vi "Test_Echo_Send_Report.vi"() -> ()   [LabVIEW 2021]
doc: "Test of Echo_Send_Report without device: one stored echo at key 196615, two calls with the same ack. Expect one 36-byte report datagram on 127.0.0.1:report port, TX acks matched 1, unmatched acks 1."
uses:
  echo/Echo_Context.ctl
  echo/Echo_Time_Store.ctl
  echo/Echo_Frame_Kind.ctl
  echo/Echo_Frame.ctl
  echo/Echo_Counters.ctl
panel:
  out "error out":errorcluster
  out "Echo_Counters":T1
  in  "report port":u16=5302
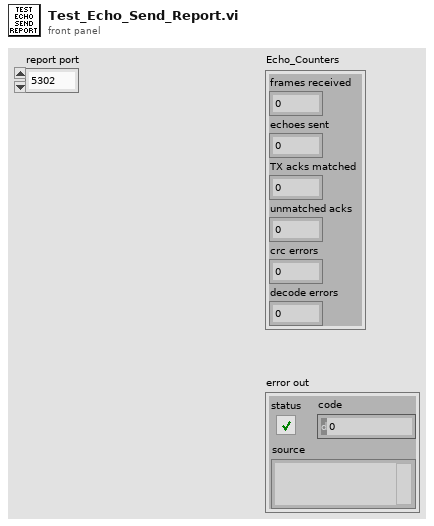
[diagram p1: front panel]
types:
  T1 = typedef "Echo_Counters.ctl" = cluster{"frames received":u32, "echoes sent":u32, "TX acks matched":u32, "unmatched acks":u32, "crc errors":u32, "decode errors":i32}
  T2 = typedef "Echo_Frame_Kind.ctl" = enum16{"Other", "Test", "Ack"}
  T3 = typedef "Echo_Frame.ctl" = cluster{"kind":T2, "id":u32, "t_dev":dbl, "seq":u16, "idx":u8, "key":i32, "index":i32}
  T4 = typedef "Echo_Time_Store.ctl" = cluster{"t_rx2_dev":dbl[], "t_rx2_lv":dbl[], "t_echo_send_lv":dbl[]}
  T5 = typedef "Echo_Context.ctl" = cluster{"TLS connection":refnum<k5>, "udp":refnum<k16>, "lv addr":u32, "report port":u16, "test lo":u32, "test hi":u32, "ack lo":u32, "ack hi":u32, "echo offset":i32}
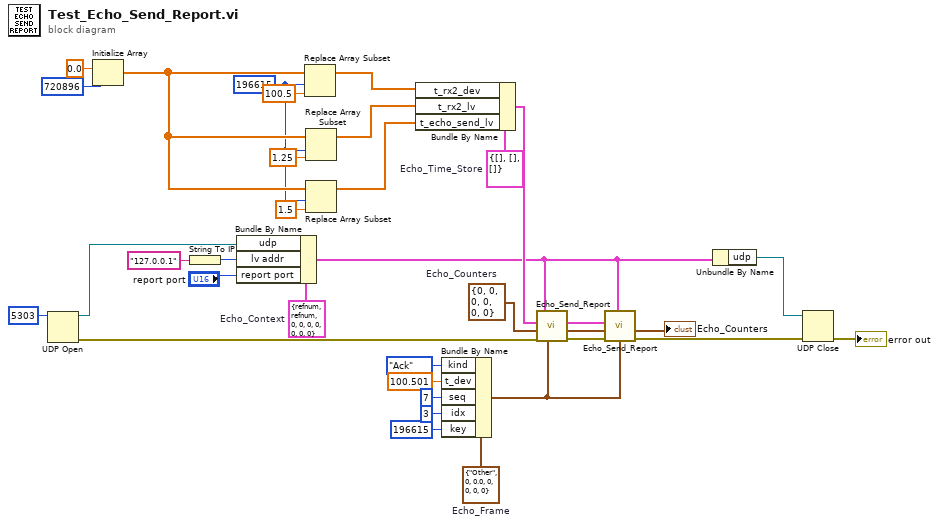
[diagram p0: block diagram]
diagram:
  w8 = T1 {"frames received"=0, "echoes sent"=0, "TX acks matched"=0, "unmatched acks"=0, "crc errors"=0, "decode errors"=0}  # Echo_Counters
  w21 = 196615 ("index")
  w33 = T3 {"kind"=enum."Other", "id"=0, "t_dev"=0.0, "seq"=0, "idx"=0, "key"=0, "index"=0}  # Echo_Frame
  w34 = T4 {"t_rx2_dev"=[], "t_rx2_lv"=[], "t_echo_send_lv"=[]}  # Echo_Time_Store
  w35 = T5 {"TLS connection"=refnum, "udp"=refnum, "lv addr"=0, "report port"=0, "test lo"=0, "test hi"=0, "ack lo"=0, "ack hi"=0, "echo offset"=0}  # Echo_Context
  n1 = UDP Open(11:u16 5303 ("port")) -> (port=w28:refnum<k16>, 0:w6:errorcluster)  [unwired: 4 in, 1 out]
  n2 = Initialize Array(0.0 ("element"), 720896 ("dimension size")) -> (w22:dbl[])
  n3 = String To IP(1:"127.0.0.1" ("name")) -> (0:w27:u32)
  n4 = Bundle By Name(cluster=w35, "udp"=w28, "lv addr"=w27, "report port"="report port") -> (w3:T5)
  n5 = Replace Array Subset(array=w22, new element=100.5 ("new element/subarray"), index=w21) -> (w17:dbl[])
  n6 = Replace Array Subset(array=w22, new element=1.25 ("new element/subarray"), index=w21) -> (w16:dbl[])
  n7 = Replace Array Subset(array=w22, new element=1.5 ("new element/subarray"), index=w21) -> (w15:dbl[])
  n8 = Bundle By Name(cluster=w34, "t_rx2_dev"=w17, "t_rx2_lv"=w16, "t_echo_send_lv"=w15) -> (w9:T4)
  n9 = Bundle By Name(cluster=w33, "kind"=Echo_Frame_Kind."Ack", "t_dev"=100.501, "seq"=u16 7, "idx"=u8 3, "key"=196615) -> (w7:T3)
  n10 = call "Echo_Send_Report.vi"("frame"=w7, "context"=w3, "error in (no error)"=w6, "counters in"=w8, "time store in"=w9) -> ("error out"=w32:errorcluster, "counters out"=w30:T1, "time store out"=w31:T4)  [unwired: 4 in]
  n11 = call "Echo_Send_Report.vi"("frame"=w7, "context"=w3, "error in (no error)"=w32, "counters in"=w30, "time store in"=w31) -> ("error out"=w4:errorcluster, "counters out"=→"Echo_Counters":T1)  [unwired: 4 in, 1 out]
  n12 = Unbundle By Name(w3) -> ("udp"=w2:refnum<k16>)
  n13 = UDP Close(connection ID=w2, 8:w4) -> (error out=→"error out":errorcluster)  [unwired: 1 out]
